vi "OwnMergeWireTerms.vi"() -> ()   [LabVIEW 2024]
panel:
  out "error out":errorcluster caption="错误输出"
  out "terminal_ids":u32[](array[numeric])
  in  "terminal_ids type":u32
  in  "wire_id":u32
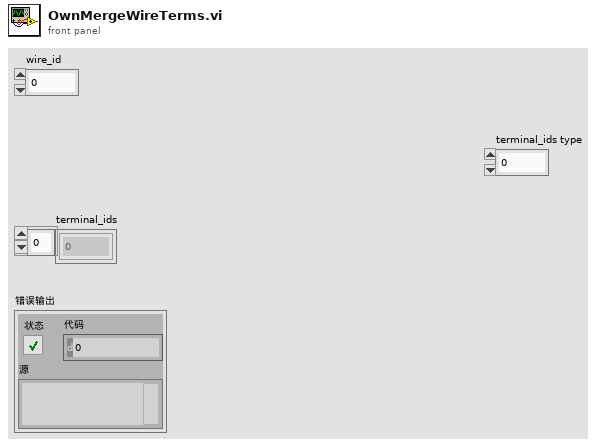
[diagram p1: front panel]
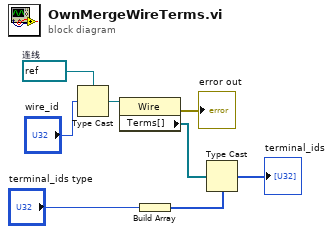
[diagram p0: block diagram]
diagram:
  w7 = refnum<vi> refnum  # 连线
  n1 = Type Cast ("强制类型转换")(type=w7, x="wire_id") -> (*(type *) &x=w6:refnum<vi>)
  n2 = property on="属性节点" class="Wire"(reference=w6) -> (error out=→"error out":errorcluster, "Terms[]"=w5:refnum<vi>[])  [unwired: 1 in, 1 out]
  n3 = Build Array ("创建数组")("terminal_ids type") -> (w3:u32[])
  n4 = Type Cast ("强制类型转换")(type=w3, x=w5) -> (*(type *) &x=→"terminal_ids":u32[])
